vi "Put file.vi"(8 "error in (no error)":errorcluster, 9 "Local path":path, 10 "Remote path":string, 11 "SCP File Transfer in":refnum<class "SCP File Transfer.lvclass">) -> (0 "error out":errorcluster, 3 "SCP File Transfer out":refnum<class "SCP File Transfer.lvclass">)   [LabVIEW 2014, in "PL Framework Configuration Tool.lvlib" / "SCP File Transfer.lvclass"]
doc: "Puts the file located at \"Local path\" at \"Remote path\". The VI also creates all needed directories if the \"Remote path\" contains directories that don't exist on the target.\n\nThe recommended file path format for \"Remote path\" is \"/directory1/directory2/file.extension\". However, the VI will accept other formats and transform the path appropriately in most cases. Use the \"Strip path.vi\" and \"Build path.vi\" VIs to help with handling remote path strings."
uses:
  SCP File Transfer.lvclass
  SCP File Transfer.lvclass/SCP File Transfer.ctl
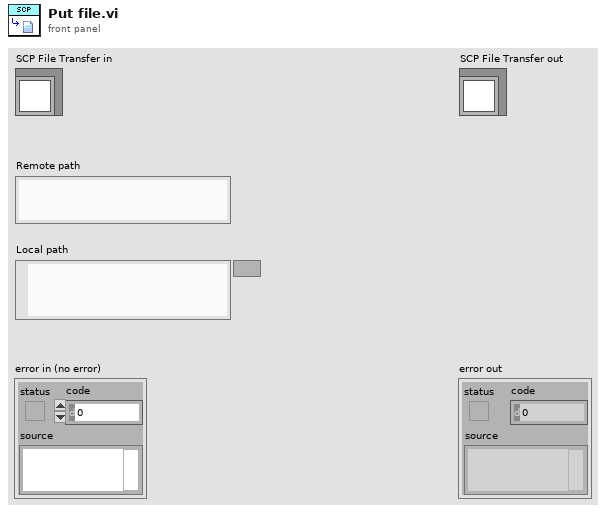
[diagram p1: front panel]
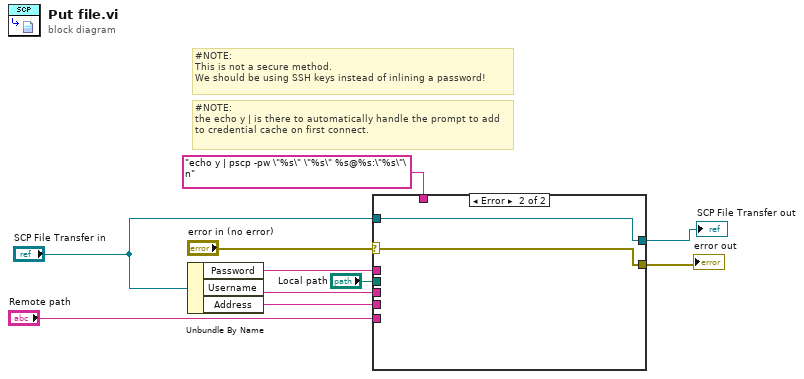
[diagram p0: block diagram]
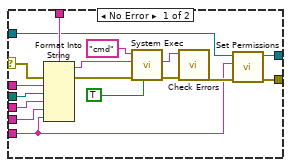
[diagram p2: hidden frame]
diagram:
  # "#NOTE:\nthe echo y | is there to automatically handle the prompt to add to credential cache on first connect."
  # "#NOTE:\nThis is not a secure method.\nWe should be using SSH keys instead of inlining a password!"
  n1 = Unbundle By Name("SCP File Transfer in") -> ("Password"=w3:string, "Username"=w8:string, "Address"=w2:string)
  n2 = case shown="Error" "error in (no error)" {
    selector: "error in (no error)" -> [w11 w28]
    tunnel: "echo y | pscp -pw \"%s\" \"%s\" %s@%s:\"%s\"\n" ("format string") -> [w26 _]
    tunnel: "Local path" -> [w21 _]
    tunnel: w8 -> [w20 _]
    tunnel: [w17 w29] -> w7
    tunnel: "SCP File Transfer in" -> [w16 w29]
    tunnel: "Remote path" -> [w15 _]
    tunnel: [w14 w28] -> w4
    tunnel: w3 -> [w13 _]
    tunnel: w2 -> [w12 _]
    frame No Error {
      n3 = Format Into String(format string=w26, error in=w11, w13, w21, w20, w12, w15) -> (resulting string=w22:string, error out=w27:errorcluster)  [unwired: 1 in]
      n4 = call <vilib>:"System Exec.vi"("run minimized? (F)"=TRUE, "error in (no error)"=w27, "standard input"=w22, "command line"="cmd") -> ("error out"=w23:errorcluster, "standard error"=w24:string)  [unwired: 4 in, 2 out]
      n5 = call "Check Errors.vi"("error in (no error)"=w23, "standard error"=w24) -> ("error out"=w18:errorcluster)  [unwired: 9 in]
      n6 = call "Set Permissions.vi"("error in (no error)"=w18, "Remote path"=w15, "SCP File Transfer in"=w16) -> ("error out"=w14:errorcluster, "SCP File Transfer out"=w17:refnum<class "SCP File Transfer.lvclass">)  [unwired: 7 in]
    }
    frame Error {
    }
  }
  "error out" <- w4
  "SCP File Transfer out" <- w7
